vi "Rainbow.vi"() -> ()   [LabVIEW 2026]
panel:
  out "Current Color":string
  in  "Stop":bool
  in  "Next":bool
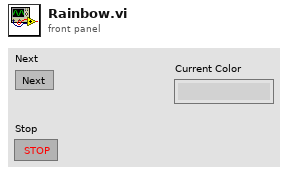
[diagram p1: front panel]
types:
  T1 = enum16{"Red", "Orange", "Yellow", "Green", "Blue", "Indigo", "Violet"}
  T2 = enum16{"Show Color", "Wait", "Next Color", "Stop"}
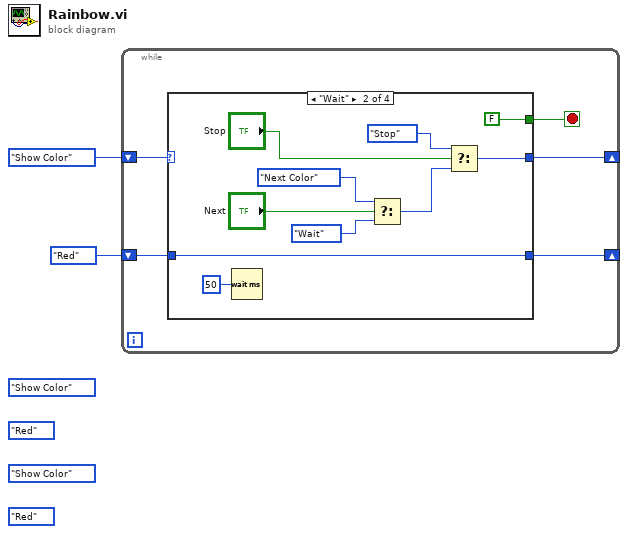
[diagram p0: block diagram]
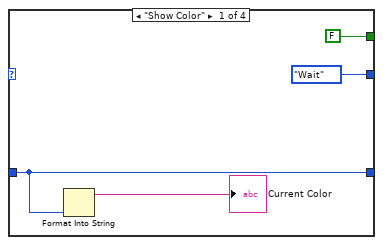
[diagram p2: hidden frame]
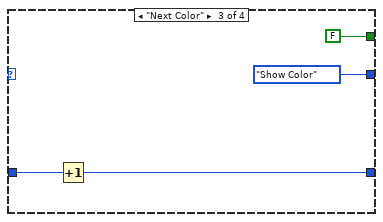
[diagram p3: hidden frame]
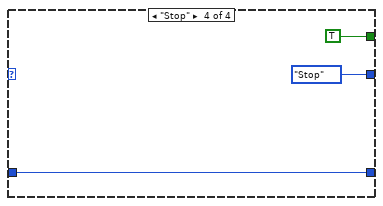
[diagram p4: hidden frame]
diagram:
  (unwired) T1."Red" ("Color")
  (unwired) T2."Show Color" ("State")
  (unwired) T1."Red" ("Color")
  (unwired) T2."Show Color" ("State")
  n1 = while {
    shift-right: [w4] -> _
    shift-left: T2."Show Color" ("State") -> [w7]
    shift-right: [w5] -> _
    shift-left: T1."Red" ("Color") -> [w6]
    stop <- w3 stop-if-true
    n2 = case shown="\"Wait\"" w7 {
      tunnel: w6 -> [w11 w21 w25 w28]
      tunnel: [w11 w21 w24 w28] -> w5
      tunnel: [T2."Wait" ("State") w13 T2."Show Color" ("State") T2."Stop" ("State")] -> w4
      tunnel: [FALSE FALSE FALSE TRUE] -> w3
      frame "Show Color" {
        n3 = Format Into String(w11) -> (resulting string=→"Current Color":string)  [unwired: 3 in, 1 out]
      }
      frame "Wait" {
        n4 = Wait (ms)(milliseconds to wait=50) -> ()  [unwired: 1 out]
        n5 = Select(t=T2."Next Color" ("State"), s="Next", f=T2."Wait" ("State")) -> (s? t:f=w14:T2)
        n6 = Select(t=T2."Stop" ("State"), s="Stop", f=w14) -> (s? t:f=w13:T2)
      }
      frame "Next Color" {
        n7 = Increment(x=w25) -> (x+1=w24:T1)
      }
      frame "Stop" {
      }
    }
  }
